vi "tag bus to wire.vi"(7 "unique key":string, 8 "error in":errorcluster, 11 "data table in":T1) -> (0 "error out":errorcluster, 1 "data offset":i32, 2 "wire data":string, 3 "data table out":T1)   [LabVIEW 2013, in "TEC runtime.lvclass"]
uses:
  TEC runtime.lvclass
  <vilib>/NI/Tag Bus/table/data table.ctl
  <vilib>/NI/Tag Bus/table/data table.lvlib
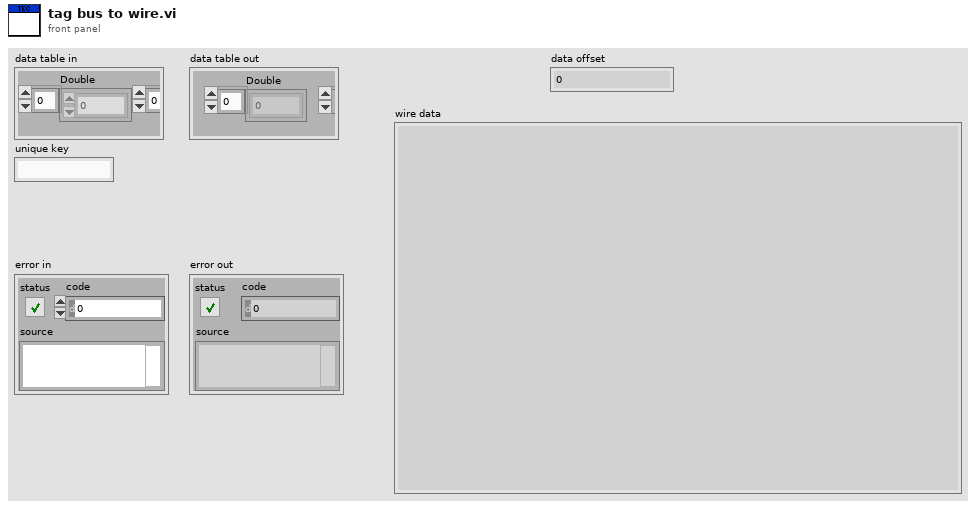
[diagram p1: front panel]
types:
  T1 = typedef "tag bus.lvlib/data table.lvlib/data table.ctl" = cluster{"Double":dbl[], "Single":sgl[], "I64":i64[], "I32":i32[], "I16":i16[], "I8":i8[], "U64":u64[], "U32":u32[], "U16":u16[], "U8":u8[], "Boolean":bool[], "String":string[], "Array of Double":cluster{"DBL Array":dbl[]}[], "Array of Single":cluster{"SGL Array":sgl[]}[], "Array of I64":cluster{"I64 Array":i64[]}[], "Array of I32":cluster{"I32 Array":i32[]}[], "Array of I16":cluster{"I16 Array":i16[]}[], "Array of I8":cluster{"I8 Array":i8[]}[], "Array of U64":cluster{"U64 Array":u64[]}[], "Array of U32":cluster{"U32 Array":u32[]}[], "Array of U16":cluster{"U16 Array":u16[]}[], "Array of U8":cluster{"U8 Array":u8[]}[], "Array of Boolean":cluster{"Boolean Array":bool[]}[], "Array of String":cluster{"String Array":string[]}[]}
  T2 = enum16{"big-endian, network order", "native, host order", "little-endian"}
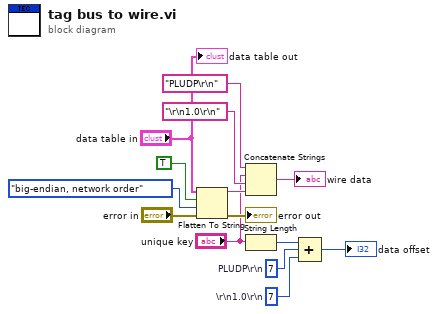
[diagram p0: block diagram]
diagram:
  w2 = 7  # \r\n1.0\r\n
  w3 = 7  # PLUDP\r\n
  n1 = Flatten To String(anything="data table in", prepend array or string size? (T)=TRUE, byte order (0:big-endian, network order)=T2."big-endian, network order", error in (no error)="error in") -> (data string=w10:string, error out=→"error out":errorcluster)  [unwired: 1 out]
  n2 = Concatenate Strings("PLUDP\r\n" ("string"), "unique key", "\r\n1.0\r\n" ("string"), w10) -> (→"wire data":string)
  n3 = String Length(string="unique key") -> (length=w4:i32)
  n4 = Compound Arithmetic op=ADD(w4, w3, w2) -> (→"data offset":i32)
  "data table out" <- "data table in"
